vi "Config_Path_G.vi"(8 "error in (no error)":errorcluster caption="错误输入（无错误）", 10 "pattern":string="AA-Path_config.xlsx") -> (0 "error out":errorcluster caption="错误输出", 2 "路径":path)   [LabVIEW 2025, in "Path_management.lvclass"]
uses:
  Path_management.lvclass
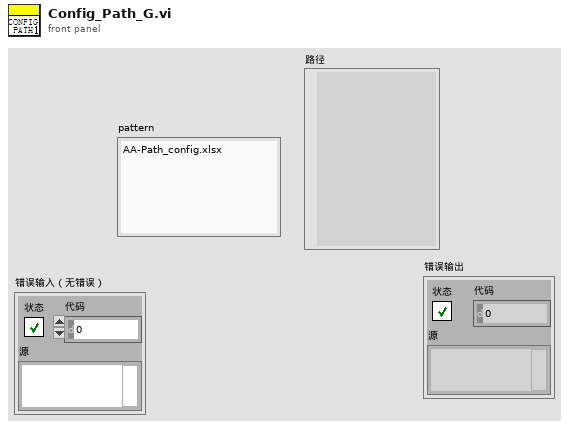
[diagram p1: front panel]
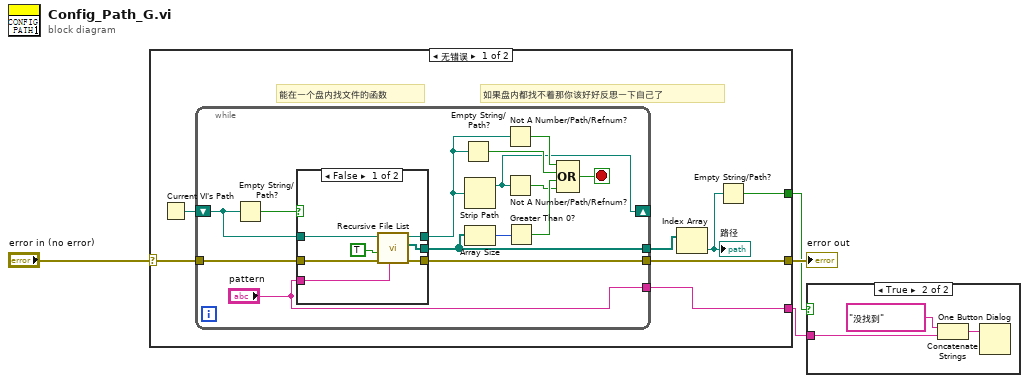
[diagram p0: block diagram]
diagram:
  n1 = case shown="无错误" "error in (no error)" {
    selector: "error in (no error)" -> [w10 w33]
    tunnel: [w11 w33] -> w2
    tunnel: [w7 _] -> w3
    tunnel: [w5 _] -> w1
    frame No Error {
      # "如果盘内都找不着那你该好好反思一下自己了"
      # "能在一个盘内找文件的函数"
      n2 = Current VI's Path() -> (path=w9:path)
      n3 = while {
        shift-right: [w17] -> _
        shift-left: w9 -> [w13]
        tunnel: [w19] -> w8
        tunnel: [w14] -> w11
        tunnel: w10 -> [w18]
        tunnel: ["pattern"] -> w7
        stop <- w21 stop-if-true
        n4 = Empty String/Path?(string/path=w13) -> (empty?=w12:bool)
        n5 = case shown="False" w12 {
          tunnel: [w32 _] -> w20
          tunnel: [w31 _] -> w19
          tunnel: w13 -> [w30 _]
          tunnel: w18 -> [w29 _]
          tunnel: "pattern" -> [w27 _]
          tunnel: [w26 _] -> w14
          frame False {
            n6 = call <vilib>:"Recursive File List.vi"("pattern"=w27, "error in (no error)"=w29, "Continue Recursing on Error? (F)"=TRUE ("Treat LLBs as Folders?"), "Folder Path"=w30) -> ("error out"=w26:errorcluster, "All Files in Dir"=w31:path[], "dup Folder Path"=w32:path)  [unwired: 1 in, 4 out]
          }
          frame True {
          }
        }
        n7 = Empty String/Path?(string/path=w20) -> (empty?=w23:bool)
        n8 = Strip Path(path=w20) -> (stripped path=w17:path)  [unwired: 1 out]
        n9 = Array Size(array=w19) -> (size(s)=w25:i32)
        n10 = Not A Number/Path/Refnum?(number/path/refnum=w20) -> (NaN/Path/Refnum?=w24:bool)
        n11 = Not A Number/Path/Refnum?(number/path/refnum=w17) -> (NaN/Path/Refnum?=w16:bool)
        n12 = Greater Than 0?(x=w25) -> (x > 0?=w22:bool)
        n13 = Compound Arithmetic op=OR(w24, w23, w22, w16) -> (w21:bool)
      }
      n14 = Index Array(array=w8) -> (element=w6:path)  [unwired: 1 in]
      "路径" <- w6
      n15 = Empty String/Path?(string/path=w6) -> (empty?=w5:bool)
    }
    frame Error {
    }
  }
  "error out" <- w2
  n16 = case shown="True" w1 {
    tunnel: w3 -> [_ w34]
    frame False {
    }
    frame True {
      n17 = Concatenate Strings("没找到" ("消息"), w34) -> (w35:string)
      n18 = One Button Dialog(message=w35) -> ()  [unwired: 1 in, 1 out]
    }
  }
